vi "Read File dialog event.vi"(8 "error in (no error)":errorcluster, 11 "Scope5782_six_channel in":refnum<class "Scope5782_six_channel.lvclass">) -> (0 "error out":errorcluster, 2 "File dialog event":T1, 3 "Scope5782_six_channel out":refnum<class "Scope5782_six_channel.lvclass">)   [LabVIEW 2025, in "Scope5782_six_channel.lvclass"]
uses:
  Scope5782_six_channel.lvclass
  Scope5782_six_channel.lvclass/Scope5782_six_channel.ctl
  Utilities/FileDialogResult.ctl
  Utilities/FileDialogEvent.ctl
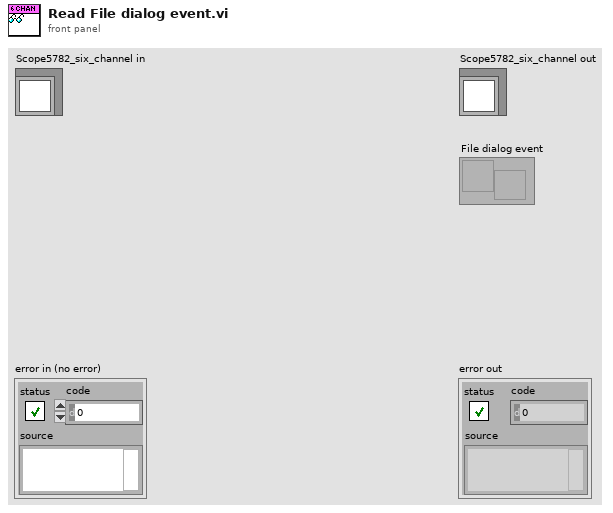
[diagram p1: front panel]
types:
  T1 = typedef "FileDialogEvent.ctl" = refnum<user-event>
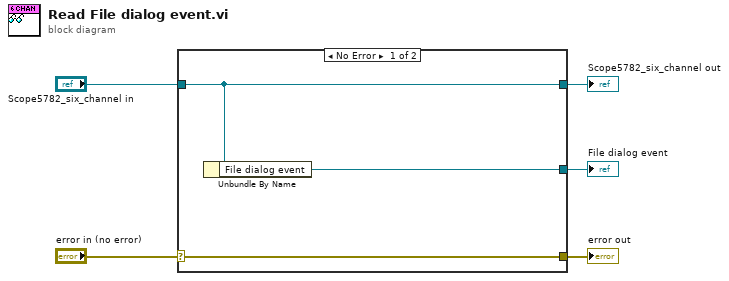
[diagram p0: block diagram]
diagram:
  n1 = case shown="No Error" "error in (no error)" {
    selector: "error in (no error)" -> [w8 w9]
    tunnel: [w8 w9] -> w4
    tunnel: [w7 w10] -> w2
    tunnel: "Scope5782_six_channel in" -> [w7 w10]
    tunnel: [w6 _] -> w1
    frame No Error {
      n2 = Unbundle By Name(w7) -> ("File dialog event"=w6:T1)
    }
    frame Error {
    }
  }
  "error out" <- w4
  "Scope5782_six_channel out" <- w2
  "File dialog event" <- w1
